vi "UE_Feedback_Freshness.vi"(3 "max_age_ms":dbl, 4 "sample_ms":dbl, 5 "now_ms":dbl) -> (1 "fresh":bool, 2 "age_ms":dbl)   [LabVIEW 2026]
doc: "INTENT: Measure feedback age using monotonic clock and check nonnegative age not exceeding maximum. INPUTS: now_ms (double), sample_ms (double), max_age_ms (double). OUTPUTS: age_ms (double), fresh (bool). DESIGN CONSTRAINT: Clocks must share one monotonic domain; sample validity is separately checked. REQUIREMENTS: SRS-F-022. No physical hardware side effects. Acceptance requires native LabVIEW compilation and behavioral testing."
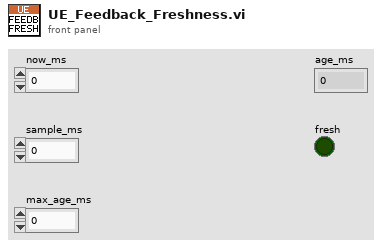
[diagram p1: front panel]
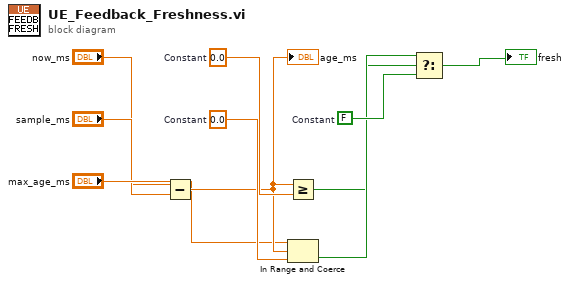
[diagram p0: block diagram]
diagram:
  w9 = FALSE  # Constant
  w7 = 0.0  # Constant
  w5 = 0.0  # Constant
  n1 = Subtract(x="now_ms", y="sample_ms") -> (x-y=w4:dbl)
  "age_ms" <- w4
  n2 = Greater Or Equal?(x=w4, y=w5) -> (x >= y?=w6:bool)
  n3 = In Range and Coerce(upper limit="max_age_ms", x=w4, lower limit=w7) -> (In Range?=w8:bool)  [unwired: 1 out]
  n4 = Select(t=w8, s=w6, f=w9) -> (s? t:f=→"fresh":bool)
